vi "Evaluate.vi"(8 "error in (no error)":errorcluster, 11 "One or More In":refnum<class "One or More.lvclass">) -> (0 "error out":errorcluster, 1 "Message":string, 2 "Passed?":bool)   [LabVIEW 2020, in "One or More.lvlib" / "One or More.lvclass"]
uses:
  One or More.lvclass
  One or More.lvclass/One or More.ctl
  Core/VI Call/VI Call.lvclass
  Core/Comparator/Comparator.lvclass
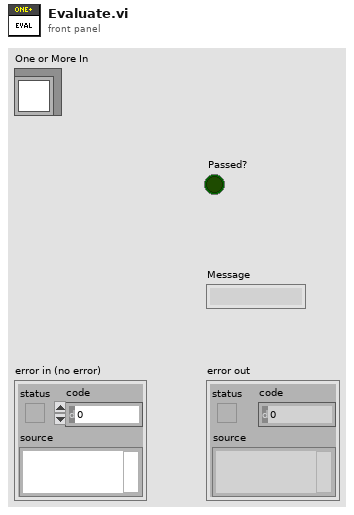
[diagram p1: front panel]
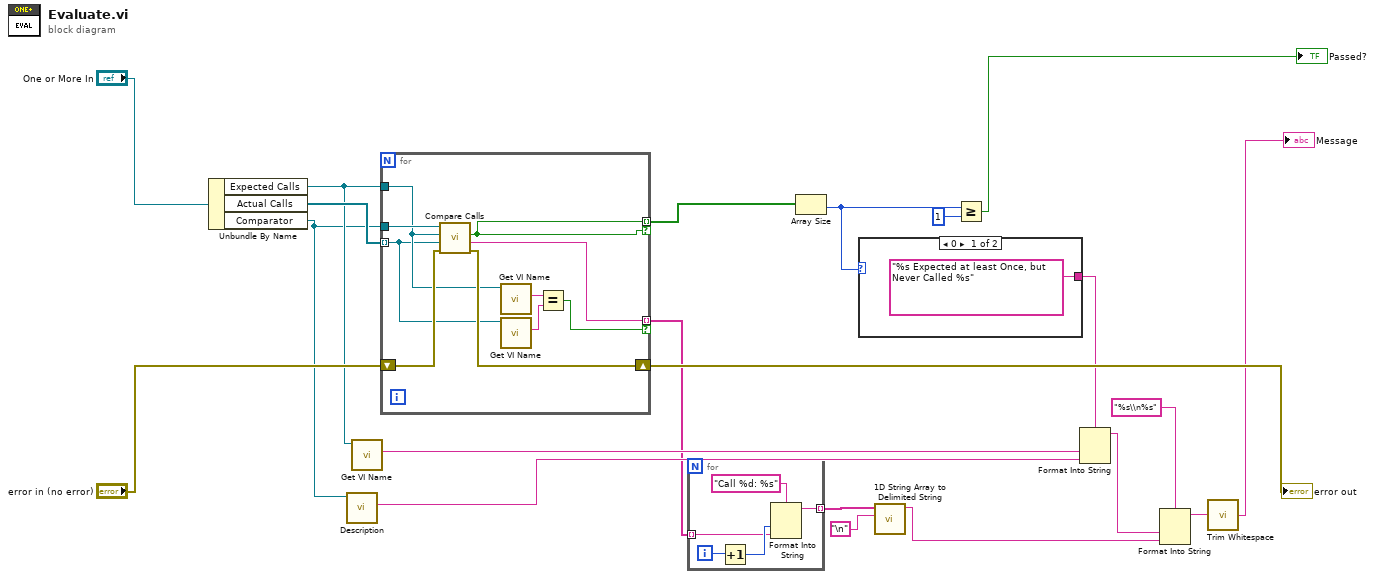
[diagram p0: block diagram]
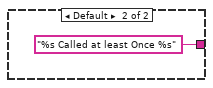
[diagram p2: hidden frame]
diagram:
  n1 = Unbundle By Name("One or More In") -> ("Expected Calls"=w12:refnum<class "VI Call.lvclass">, "Actual Calls"=w18:refnum<class "VI Call.lvclass">[], "Comparator"=w11:refnum<class "Comparator.lvclass">)
  n2 = call-dynamic "Description.vi"("Comparator in"=w11) -> ("Description"=w14:string)  [unwired: 9 in, 1 out]
  n3 = call-dynamic "Get VI Name.vi"("VI Call In"=w12) -> ("VI Name"=w13:string)  [unwired: 9 in, 1 out]
  n4 = for {
    tunnel: w12 -> [w23]
    tunnel: w11 -> [w31]
    tunnel: w18 -> [w22] mode=indexing
    shift-right: [w29] -> w16
    shift-left: "error in (no error)" -> [w30]
    tunnel: [w28] -> w20 mode=indexing if=w28
    tunnel: [w27] -> w1 mode=indexing if=w24
    n5 = call-dynamic "Compare Calls.vi"("error in (no error)"=w30, "VI Call 2"=w22, "VI Call 1"=w23, "Comparator in"=w31) -> ("error out"=w29:errorcluster, "Description"=w27:string, "Equal?"=w28:bool)  [unwired: 5 in]
    n6 = call-dynamic "Get VI Name.vi"("VI Call In"=w23) -> ("VI Name"=w26:string)  [unwired: 9 in, 1 out]
    n7 = call-dynamic "Get VI Name.vi"("VI Call In"=w22) -> ("VI Name"=w25:string)  [unwired: 9 in, 1 out]
    n8 = Equal?(x=w26, y=w25) -> (x = y?=w24:bool)
  }
  "error out" <- w16
  n9 = for {
    tunnel: w1 -> [w33] mode=indexing
    tunnel: [w32] -> w2 mode=indexing
    i -> [w35]
    n10 = Increment(x=w35) -> (x+1=w34:i32)
    n11 = Format Into String(format string="Call %d: %s", w34, w33) -> (resulting string=w32:string)  [unwired: 2 in, 1 out]
  }
  n12 = Array Size(array=w20) -> (size(s)=w10:i32)
  n13 = case shown="0" w10 {
    tunnel: ["%s Expected at least Once, but Never Called %s" ("Message") "%s Called at least Once %s" ("Message")] -> w9
    frame 0 {
    }
    frame Default {
    }
  }
  n14 = call <vilib>:"1D String Array to Delimited String.vi"("delimiter"="\n", "string array"=w2) -> ("delimited string"=w4:string)  [unwired: 9 in]
  n15 = Greater Or Equal?(x=w10, y=1) -> (x >= y?=→"Passed?":bool)
  n16 = Format Into String(format string=w9, w13, w14) -> (resulting string=w3:string)  [unwired: 2 in, 1 out]
  n17 = Format Into String(format string="%s\\n%s", w3, w4) -> (resulting string=w7:string)  [unwired: 2 in, 1 out]
  n18 = call <vilib>:"Trim Whitespace.vi"("string"=w7) -> ("trimmed string"=→"Message":string)  [unwired: 1 in]
